vi "Programatic Scroll.vi"(8 "error in":errorcluster, 9 "Pause? (F)":bool, 10 "Table Ref":refnum<vi>, 11 "Trace":string[][](table)=[["", "", "", "", ""], ["", "", "", "", ""], ["", "", "", "", ""], ["", "", "", "", ""], ["", "", "", "", ""], ["", "", "", "", ""]]) -> (0 "error out":errorcluster)   [LabVIEW 2025, in "CAN-LIN Raw Bus Capture UI.lvlib"]
doc: "Scroll the table programatically to the end (only necessary when it is unpaused, paused table will not get new data). This vi does this scrolling only when it is not paused."
uses:
  CAN-LIN Raw Bus Capture UI.lvlib
  <vilib>/Utility/miscctls.llb/LVRowAndColumnUnsignedTypeDef.ctl
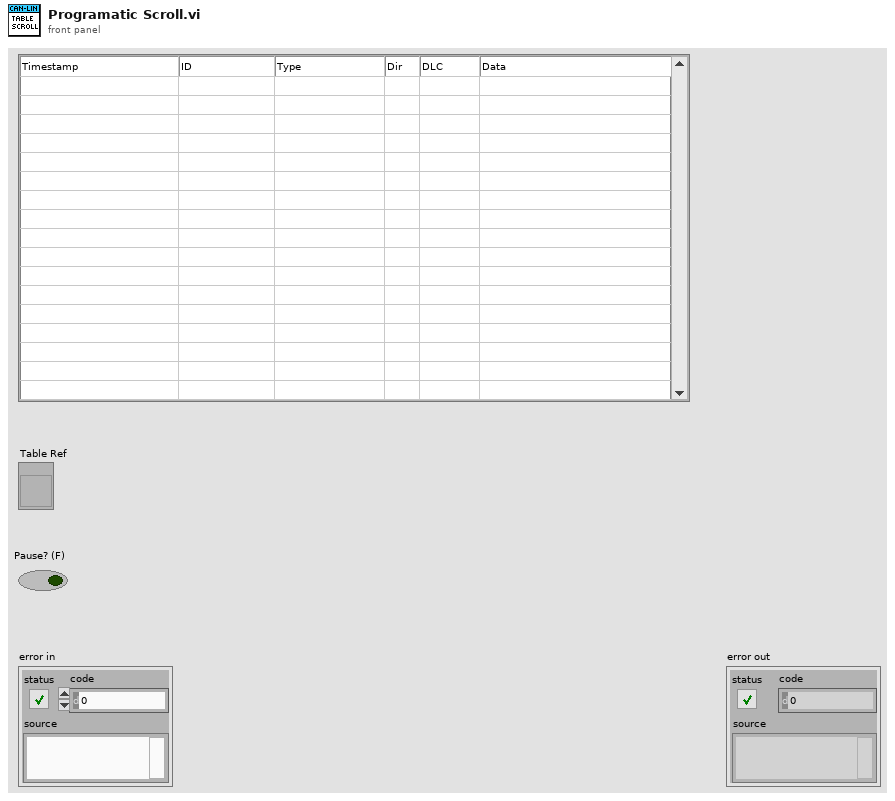
[diagram p1: front panel]
types:
  T1 = typedef "LVRowAndColumnUnsignedTypeDef.ctl" = cluster{"Row":u32, "Column":u32}
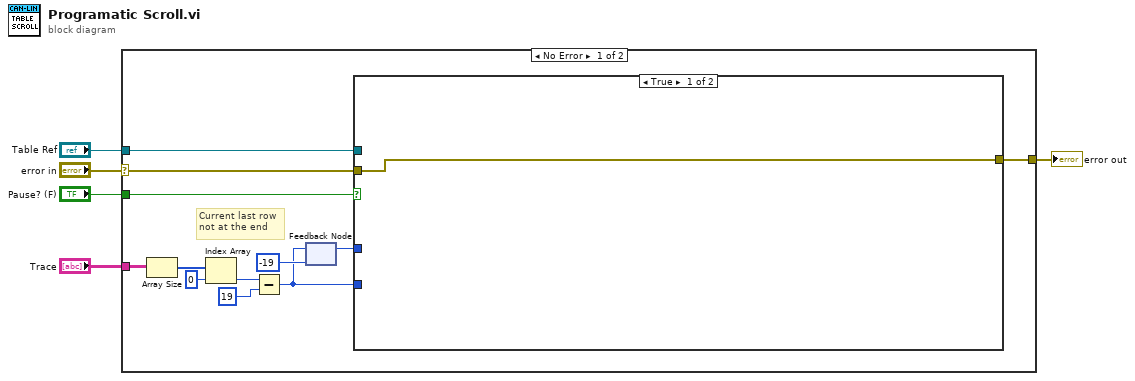
[diagram p0: block diagram]
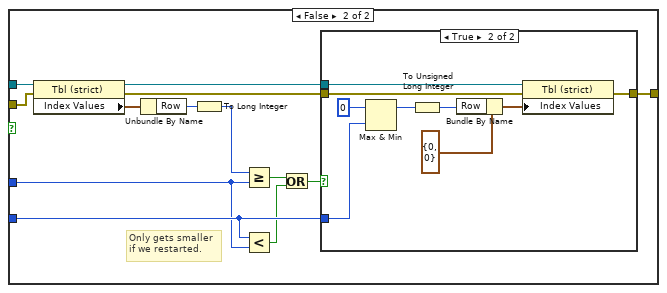
[diagram p2: hidden frame]
diagram:
  n1 = case shown="No Error" "error in" {
    selector: "error in" -> [w9 w42]
    tunnel: "Table Ref" -> [w16 _]
    tunnel: "Trace" -> [w11 _]
    tunnel: [w17 w42] -> w3
    tunnel: "Pause? (F)" -> [w6 _]
    frame No Error {
      # "Current last row\nnot at the end"
      n2 = Array Size(array=w11) -> (size(s)=w14:i32[])
      n3 = Index Array(array=w14, index=0) -> (element=w15:i32)
      n4 = Subtract(x=w15, y=19 ("max(x,y)")) -> (x-y=w8:i32)
      n5 = feedback #1(-19 ("max(x,y)")) -> (w7:i32)
      n6 = feedback-in #1(w8) -> ()
      n7 = case shown="True" w6 {
        tunnel: [w18 w31] -> w17
        tunnel: w16 -> [_ w30]
        tunnel: w9 -> [w18 w25]
        tunnel: w8 -> [_ w23]
        tunnel: w7 -> [_ w22]
        frame True {
        }
        frame False {
          # "Only gets smaller\nif we restarted."
          n8 = property on="Property Node" class="Tbl (strict)"(reference=w30, error in=w25) -> (reference out=w29:refnum<vi>, error out=w19:errorcluster, "Index Values"=w28:T1)
          n9 = Unbundle By Name(w28) -> ("Row"=w26:u32)
          n10 = To Long Integer(number=w26) -> (32bit integer=w27:i32)
          n11 = Greater Or Equal?(x=w27, y=w22) -> (x >= y?=w24:bool)
          n12 = Less?(x=w23, y=w22) -> (x < y?=w21:bool)
          n13 = Or(x=w24, y=w21) -> (x .or. y?=w20:bool)
          n14 = case shown="True" w20 {
            tunnel: [w32 w41] -> w31
            tunnel: w29 -> [_ w40]
            tunnel: w23 -> [_ w39]
            tunnel: w19 -> [w32 w38]
            frame False {
            }
            frame True {
              n15 = Max & Min(x=0 ("max(x,y)"), y=w39) -> (max(x,y)=w34:i32)  [unwired: 1 out]
              n16 = To Unsigned Long Integer(number=w34) -> (unsigned 32bit integer=w33:u32)
              n17 = Bundle By Name(cluster=T1 {"Row"=0, "Column"=0} ("Index Values"), "Row"=w33) -> (w36:T1)
              n18 = property on="Property Node" class="Tbl (strict)"(reference=w40, error in=w38, "Index Values"=w36) -> (error out=w41:errorcluster)  [unwired: 1 out]
            }
          }
        }
      }
    }
    frame Error {
    }
  }
  "error out" <- w3
